vi "Test Mixer.vi"(8 "error in (no error)":errorcluster, 11 "DSP.lvclass":refnum<class "DSP.lvclass">) -> (0 "error out":errorcluster, 3 "DSP.lvclass":refnum<class "DSP.lvclass">)   [LabVIEW 2019, in "Tests.DSP.lvlib"]
uses:
  src/DSP/DSP.lvclass
  src/DSP/Typedefs/REF.Channel--Cluster--Array.ctl
  src/DSP/Typedefs/REF.Channel--Cluster.ctl
  src/DSP/Typedefs/AI.Channel--Cluster--Array.ctl
  src/DSP/Typedefs/AI.Channel--Cluster.ctl
  src/DSP/Typedefs/DSP.Config.Timing--Cluster.ctl
  src/DSP/DSP.lvclass/DSP.ctl
  Tests.DSP.lvlib
  <vilib>/measure/NI_MABase.lvlib
panel:
  in  "AI Channels":T1=[{"Enable?"=TRUE, "Channel"=1, "References"=[1], "reference index"=0}] {"reference index" min=1; "References" items=["", "1", "2", "3"]; "Channel" min=1}
  out "Waveform Chart":dbl[](graph)
  out "key":string="AI1.Ref1.X"
  in  "index":i32=2
  out "phase out":dbl[](array[numeric])=[324.00000000000387, 61.19999999999811]
  out "Waveform 2":waveform(dbl)[](graph)
  in  "frequency":dbl[](array[numeric])=[13.0, 9.9] format="%0.2p"
  in  "REF Channels 2":T3=[{"Enable?"=TRUE, "Channel"=1, "Frequency"=13.0, "Phase"=0.0, "TC"=0.3, "Roll-Off"=2}] {"Roll-Off" min=1; "TC" min=0.0001 format="%#_3p"; "Phase" format="%.3g"; "Frequency" min=0.0001 max=10000.0 format="%.3g"; "Channel" min=1}
  out "Waveform 1":waveform(dbl)[](graph)
  in  "stop":bool
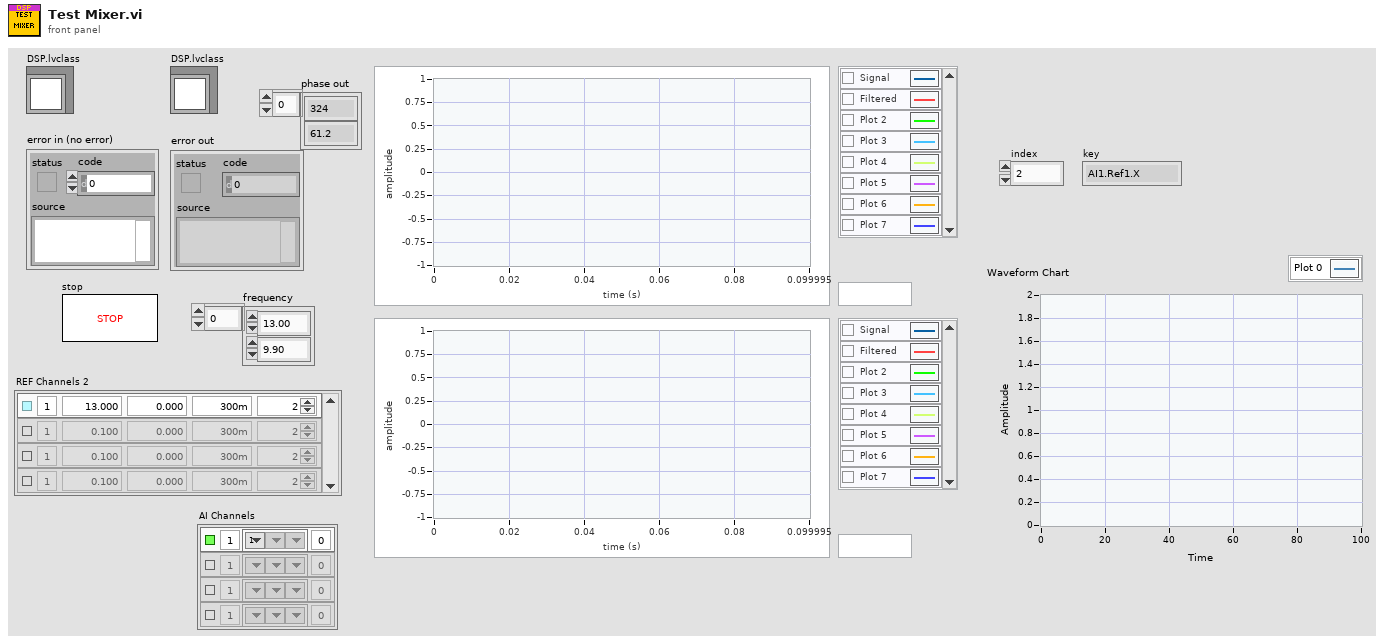
[diagram p1: front panel]
types:
  T1 = typedef "DSP.lvclass/AI.Channel--Cluster--Array.ctl" = T2[]
  T2 = typedef "DSP.lvclass/AI.Channel--Cluster.ctl" = cluster{"Enable?":bool, "Channel":i32, "References":i32[], "reference index":i32}
  T3 = typedef "DSP.lvclass/REF.Channel--Cluster--Array.ctl" = T4[]
  T4 = typedef "DSP.lvclass/REF.Channel--Cluster.ctl" = cluster{"Enable?":bool, "Channel":i32, "Frequency":dbl, "Phase":dbl, "TC":dbl, "Roll-Off":i32}
  T5 = typedef "DSP.lvclass/DSP.Config.Timing--Cluster.ctl" = cluster{"Sampling":cluster{"Fs":dbl, "#s":i32}, "Fs_Out":dbl}
  T6 = cluster{"AO":waveform(dbl)[], "AI":waveform(dbl)[], "Ref_X":waveform(dbl)[], "Ref_Y":waveform(dbl)[], "X":waveform(dbl)[], "Y":waveform(dbl)[]}
  T7 = typedef "DSP.lvclass/Results--Cluster.ctl" = cluster{"Time Stamp":timestamp, "Results (Dictionary)":T8[]}
  T8 = typedef "DSP.lvclass/Results Dictionary--Cluster.ctl" = cluster{"key":string, "value":dbl[]}
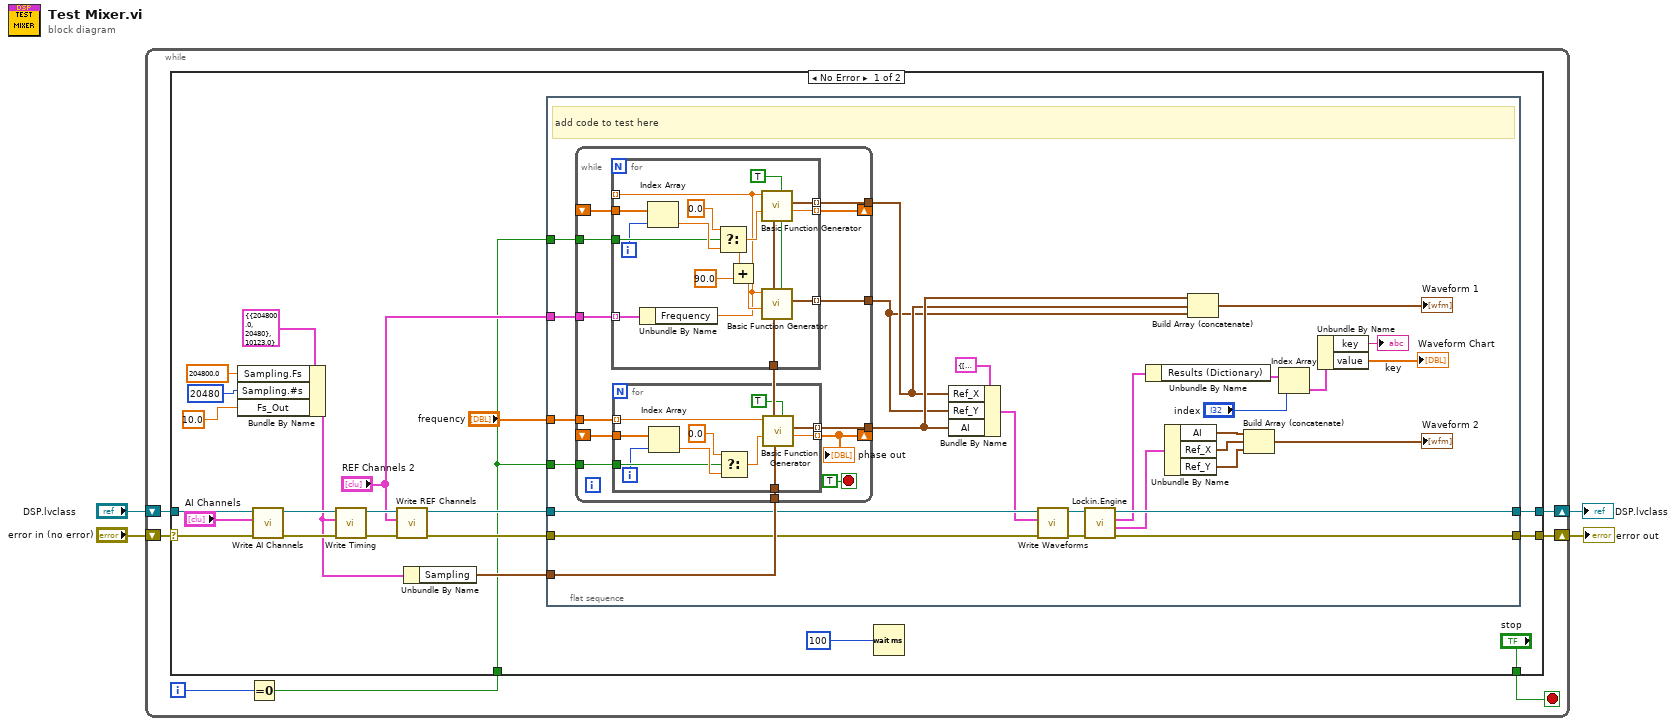
[diagram p0: block diagram]
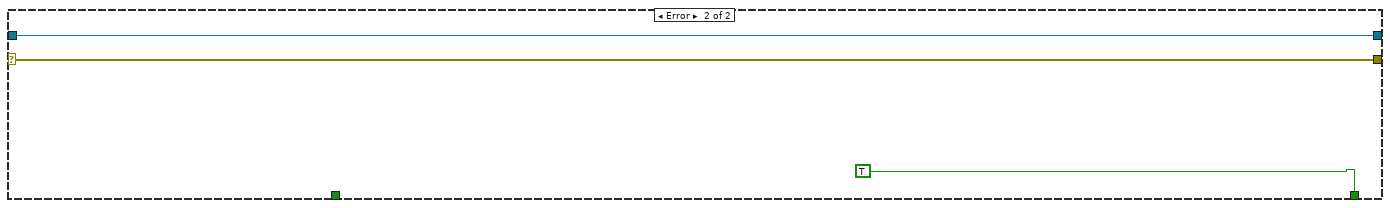
[diagram p2: hidden frame]
diagram:
  n1 = while {
    shift-right: [w10] -> w3
    shift-left: "error in (no error)" -> [w11]
    shift-right: [w8] -> w1
    shift-left: "DSP.lvclass" -> [w9]
    i -> [w7]
    stop <- w6 stop-if-true
    n2 = Equal To 0?(x=w7) -> (x = 0?=w5:bool)
    n3 = case shown="No Error" w11 {
      selector: w11 -> [w17 w103]
      tunnel: [w32 w103] -> w10
      tunnel: [w33 w102] -> w8
      tunnel: w9 -> [w15 w102]
      tunnel: ["stop" TRUE ("stop")] -> w6
      tunnel: w5 -> [w19 _]
      frame No Error {
        n4 = Bundle By Name(cluster=T5 {"Sampling"={"Fs"=204800.0, "#s"=20480}, "Fs_Out"=10123.0} ("Timing"), "Sampling.Fs"=204800.0, "Sampling.#s"=20480, "Fs_Out"=10.0) -> (w12:T5)
        n5 = call "Write AI Channels.vi"("error in (no error)"=w17, "AI Channels"="AI Channels", "DSP in"=w15) -> ("error out"=w16:errorcluster, "DSP out"=w18:refnum<class "DSP.lvclass">)  [unwired: 7 in]
        n6 = call "Write Timing.vi"("error in (no error)"=w16, "Timing"=w12, "DSP in"=w18) -> ("error out"=w26:errorcluster, "DSP out"=w27:refnum<class "DSP.lvclass">)  [unwired: 7 in]
        n7 = call "Write REF Channels.vi"("error in (no error)"=w26, "REF Channels"="REF Channels 2", "DSP in"=w27) -> ("error out"=w29:errorcluster, "DSP out"=w30:refnum<class "DSP.lvclass">)  [unwired: 7 in]
        n8 = Unbundle By Name(w12) -> ("Sampling"=w25:cluster{"Fs":dbl, "#s":i32})
        n9 = flat-sequence {
          tunnel: [w58] -> w33
          tunnel: w29 -> [w34]
          tunnel: [w57] -> w32
          tunnel: w30 -> [w38]
          tunnel: "frequency" -> [w61]
          tunnel: w25 -> [w60]
          tunnel: w19 -> [w59]
          tunnel: "REF Channels 2" -> [w56]
          tunnel: w19 -> [w55]
          frame #0 {
            # "add code to test here"
            n10 = while {
              tunnel: w61 -> [w74]
              tunnel: w60 -> [w68]
              tunnel: [w73] -> w49
              shift-right: [w72] -> _
              shift-left: _ -> [w71]
              tunnel: w59 -> [w69]
              tunnel: [w67] -> w48
              tunnel: [w66] -> w47
              shift-right: [w65] -> _
              shift-left: _ -> [w64]
              tunnel: w56 -> [w63]
              tunnel: w55 -> [w62]
              stop <- TRUE stop-if-true
              n11 = for {
                tunnel: [w89] -> w67 mode=indexing
                tunnel: [w75] -> _ mode=indexing
                tunnel: w68 -> [w81]
                tunnel: [w88] -> w65 mode=indexing
                tunnel: w64 -> [w87]
                tunnel: w62 -> [w84]
                tunnel: [w80] -> w66 mode=indexing
                tunnel: w63 -> [w79] mode=indexing
                i -> [w83]
                w82 = TRUE ("reset signal")
                n12 = Unbundle By Name(w79) -> ("Frequency"=w75:dbl)
                n13 = Index Array(array=w87, index=w83) -> (element=w85:dbl)
                n14 = Select(t=0.0, s=w84, f=w85) -> (s? t:f=w78:dbl)
                n15 = Add(x=w78, y=90.0) -> (x+y=w76:dbl)
                n16 = call <vilib>:"Basic Function Generator.vi"("reset signal"=w82, "sampling info"=w81, "phase"=w78, "frequency"=w75) -> ("phase out"=w88:dbl, "signal out"=w89:waveform(dbl))  [unwired: 5 in, 1 out]
                n17 = call <vilib>:"Basic Function Generator.vi"("reset signal"=w82, "sampling info"=w81, "phase"=w76, "frequency"=w75) -> ("signal out"=w80:waveform(dbl))  [unwired: 5 in, 2 out]
              }
              n18 = for {
                tunnel: [w100] -> w73 mode=indexing
                tunnel: w74 -> [w99] mode=indexing
                tunnel: w68 -> [w98]
                tunnel: [w97] -> w72 mode=indexing
                tunnel: w71 -> [w96]
                tunnel: w69 -> [w91]
                i -> [w90]
                n19 = Index Array(array=w96, index=w90) -> (element=w93:dbl)
                n20 = Select(t=0.0, s=w91, f=w93) -> (s? t:f=w94:dbl)
                n21 = call <vilib>:"Basic Function Generator.vi"("reset signal"=TRUE, "sampling info"=w98, "phase"=w94, "frequency"=w99) -> ("phase out"=w97:dbl, "signal out"=w100:waveform(dbl))  [unwired: 5 in, 1 out]
              }
              "phase out" <- w72
            }
            n22 = Bundle By Name(cluster=T6 {"AO"=[], "AI"=[], "Ref_X"=[], "Ref_Y"=[], "X"=[], "Y"=[]} ("Waveforms"), "Ref_X"=w48, "Ref_Y"=w47, "AI"=w49) -> (w37:T6)
            n23 = call "Write Waveforms.vi"("error in (no error)"=w34, "Waveforms"=w37, "DSP in"=w38) -> ("error out"=w35:errorcluster, "DSP out"=w36:refnum<class "DSP.lvclass">)  [unwired: 7 in]
            n24 = call "Lockin.Engine.vi"("error in (no error)"=w35, "DSP in"=w36) -> ("error out"=w57:errorcluster, "Downsampled Waveforms"=w54:T6, "Results"=w45:T7, "DSP out"=w58:refnum<class "DSP.lvclass">)  [unwired: 5 in, 1 out]
            n25 = Unbundle By Name(w45) -> ("Results (Dictionary)"=w44:T8[])
            n26 = Unbundle By Name(w54) -> ("AI"=w51:waveform(dbl)[], "Ref_X"=w53:waveform(dbl)[], "Ref_Y"=w52:waveform(dbl)[])
            n27 = Build Array (concatenate)(w49, w48, w47) -> (→"Waveform 1":waveform(dbl)[])
            n28 = Build Array (concatenate)(w51, w53, w52) -> (→"Waveform 2":waveform(dbl)[])
            n29 = Index Array(array=w44, index="index") -> (element=w42:T8)
            n30 = Unbundle By Name(w42) -> ("key"=→"key":string, "value"=→"Waveform Chart":dbl[])
          }
        }
        n31 = Wait (ms)(milliseconds to wait=u32 100) -> ()  [unwired: 1 out]
      }
      frame Error {
      }
    }
  }
  "error out" <- w3
  "DSP.lvclass" <- w1
